vi "W11_Alarm_TempLow.vi"() -> ()   [LabVIEW 2018]
doc: "Use this template to build a VI to use as a subVI."
panel:
  in  "stop":bool
  out "alarm lamp":bool
  out "alarm state":bool
  out "below SP-10":bool
  in  "ack":bool
  in  "setpoint C":dbl
  in  "temperature C":dbl
  # "Try: setpoint 175. Alarm below 165, recover at 168 or above. ACK clears the lamp only after recovery."
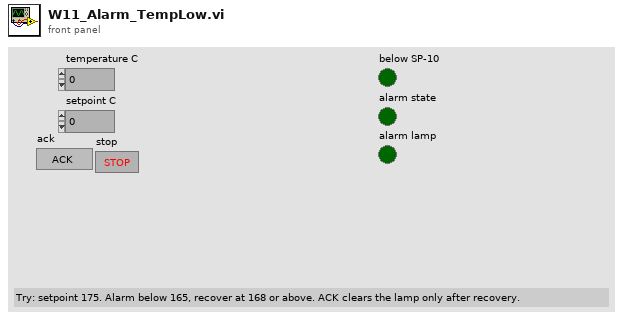
[diagram p1: front panel]
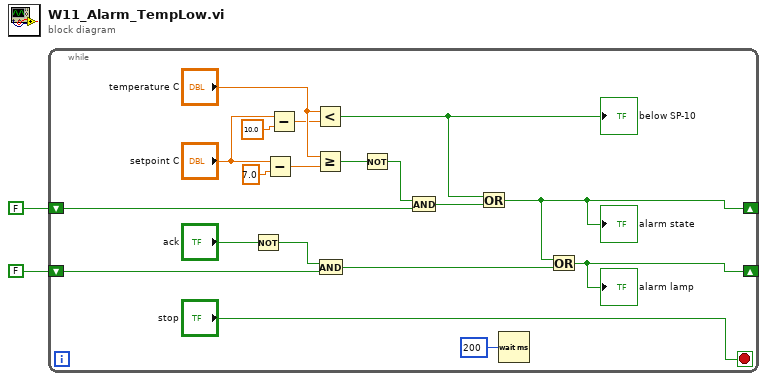
[diagram p0: block diagram]
diagram:
  n1 = while {
    shift-right: [w10] -> _
    shift-left: FALSE -> [w13]
    shift-right: [w5] -> _
    shift-left: FALSE -> [w7]
    stop <- "stop" stop-if-true
    n2 = Not(x="ack") -> (.not. x?=w8:bool)
    n3 = Subtract(x="setpoint C", y=7.0) -> (x-y=w16:dbl)
    n4 = Subtract(x="setpoint C", y=10.0) -> (x-y=w18:dbl)
    n5 = Less?(x="temperature C", y=w18) -> (x < y?=w12:bool)
    "below SP-10" <- w12
    n6 = Greater Or Equal?(x="temperature C", y=w16) -> (x >= y?=w15:bool)
    n7 = And(x=w8, y=w7) -> (x .and. y?=w6:bool)
    n8 = Not(x=w15) -> (.not. x?=w14:bool)
    n9 = And(x=w14, y=w13) -> (x .and. y?=w11:bool)
    n10 = Or(x=w12, y=w11) -> (x .or. y?=w10:bool)
    "alarm state" <- w10
    n11 = Wait (ms)(milliseconds to wait=u32 200) -> ()  [unwired: 1 out]
    n12 = Or(x=w10, y=w6) -> (x .or. y?=w5:bool)
    "alarm lamp" <- w5
  }
